vi "VIH Dialog - Find File on Disk.vi"(8 "error in":errorcluster, 9 "File Path":path, 10 "Tree Item Tag":string, 11 "Project Tree":T1) -> (0 "error out":errorcluster, 1 "New File Path":path, 2 "New Tree Item Tag":string, 3 "dup Project Tree":T1)   [LabVIEW 2014]
doc: "::: VI Helpeks :::\nCopyright (c) 2000-2026 Konstantin Shifershteyn. All rights reserved."
uses:
  VIH Project Tree Typedef - Tree Refnum.ctl
panel:
  # "VI Helpeks\nCopyright (c) 2012-2026 Konstantin Shifershteyn"
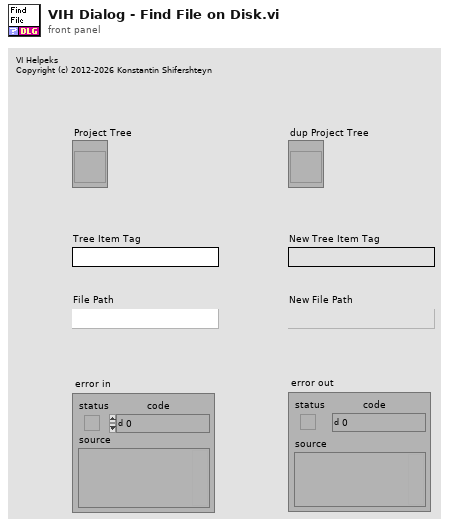
[diagram p1: front panel]
types:
  T1 = typedef "VIH Project Tree Typedef - Tree Refnum.ctl" = refnum<vi>
  T2 = cluster{"Left Button Key Shortcut":cluster{"Control":bool, "Shift":bool, "Key":string}, "Center Button Key Shortcut":cluster{"Control":bool, "Shift":bool, "Key":string}, "Right Button Key Shortcut":cluster{"Control":bool, "Shift":bool, "Key":string}}
  T3 = enum16{"Left Button", "Center Button", "Right Button", "Window Close"}
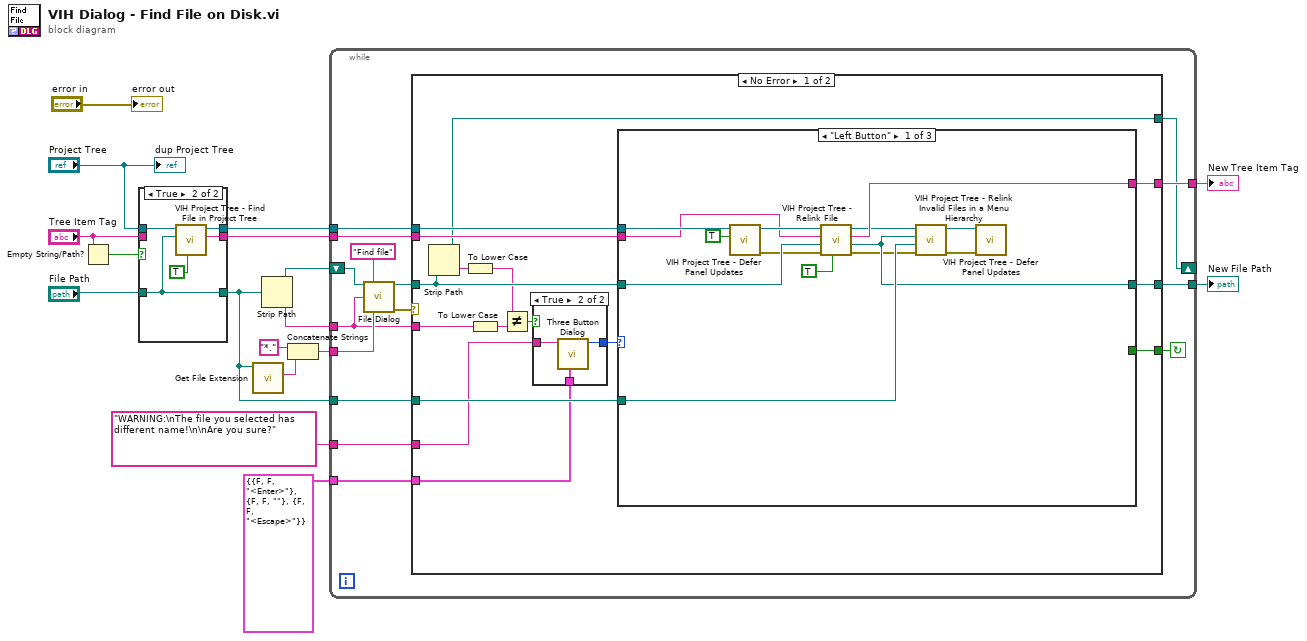
[diagram p0: block diagram]
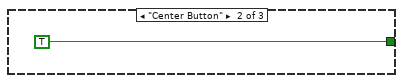
[diagram p2: hidden frame]
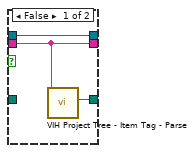
[diagram p6: hidden frame]
diagram:
  n1 = Empty String/Path?(string/path="Tree Item Tag") -> (empty?=w15:bool)
  n2 = case shown="True" w15 {
    tunnel: [w20 w24] -> w5
    tunnel: "Tree Item Tag" -> [w19 _]
    tunnel: [w19 w25] -> w14
    tunnel: "File Path" -> [_ w24]
    tunnel: "Project Tree" -> [w18 w23]
    tunnel: [w18 w21] -> w7
    frame False {
      n3 = call "VIH Project Tree - Item Tag - Parse.vi"("Tree Item Tag"=w19) -> ("Item File Path"=w20:path)  [unwired: 8 in, 2 out]
    }
    frame True {
      n4 = call "VIH Project Tree - Find File in Project Tree.vi"("Ena <Invalid> (F)"=TRUE, "File Path"=w24, "Project Tree"=w23) -> ("Tree Item Tag (Static)"=w25:string, "dup Project Tree"=w21:T1)  [unwired: 5 in, 2 out]
    }
  }
  n5 = call <vilib>:"Get File Extension.vi"("file"=w5) -> ("lowercase file extension"=w2:string)  [unwired: 7 in, 3 out]
  n6 = Strip Path(path=w5) -> (stripped path=w1:path, name=w3:string)
  n7 = Concatenate Strings("*." ("string"), w2) -> (w4:string)
  n8 = while {
    tunnel: w14 -> [w37]
    tunnel: [w36] -> w11
    tunnel: [w35] -> w10
    tunnel: "WARNING:\nThe file you selected has different name!\n\nAre you sure?" ("message") -> [w34]
    tunnel: T2 {"Left Button Key Shortcut"={"Control"=FALSE, "Shift"=FALSE, "Key"="<Enter>"}, "Center Button Key Shortcut"={"Control"=FALSE, "Shift"=FALSE, "Key"=""}, "Right Button Key Shortcut"={"Control"=FALSE, "Shift"=FALSE, "Key"="<Escape>"}} ("Keyboard Shortcuts (Left is <Enter>)") -> [w33]
    tunnel: w7 -> [w32]
    tunnel: w5 -> [w30]
    tunnel: w4 -> [w29]
    tunnel: w3 -> [w28]
    shift-right: [w26] -> _
    shift-left: w1 -> [w27]
    stop <- w31 continue-if-true
    n9 = call "File Dialog"("start path"=w27, "prompt"="Find file", "default name"=w28, "pattern (all files)"=w29) -> ("selected path"=w40:path, "error out"=w39:errorcluster)  [unwired: 8 in, 2 out]
    n10 = case shown="No Error" w39 {
      tunnel: w32 -> [w56 _]
      tunnel: w37 -> [w55 _]
      tunnel: w40 -> [w51 _]
      tunnel: w30 -> [w54 _]
      tunnel: [w53 _] -> w36
      tunnel: [w52 _] -> w35
      tunnel: w28 -> [w47 _]
      tunnel: w34 -> [w45 _]
      tunnel: w33 -> [w44 _]
      tunnel: [w42 _] -> w31
      tunnel: [w41 _] -> w26
      frame No Error {
        n11 = Strip Path(path=w51) -> (stripped path=w41:path, name=w50:string)
        n12 = To Lower Case(string=w50) -> (all lower case string=w49:string)
        n13 = To Lower Case(string=w47) -> (all lower case string=w48:string)
        n14 = Not Equal?(x=w49, y=w48) -> (x != y?=w46:bool)
        n15 = case shown="True" w46 {
          tunnel: w45 -> [_ w74]
          tunnel: w44 -> [_ w73]
          tunnel: [_ w72] -> w43
          frame False {
          }
          frame True {
            n16 = call <vilib>:"Three Button Dialog.vi"("Keyboard Shortcuts (Left is <Enter>)"=w73, "message"=w74) -> ("Which Button?"=w72:T3)  [unwired: 9 in]
          }
        }
        n17 = case shown="\"Left Button\"" w43 {
          tunnel: w56 -> [w63 _ _]
          tunnel: w55 -> [w57 _ _]
          tunnel: w54 -> [w70 _ _]
          tunnel: [w68 _ _] -> w53
          tunnel: [w67 _ _] -> w52
          tunnel: w51 -> [w69 _ _]
          tunnel: [_ TRUE _] -> w42
          frame "Left Button" {
            n18 = call "VIH Project Tree - Defer Panel Updates.vi"("Defer Panel Updates (F)"=TRUE, "Project Tree"=w63) -> ("error out"=w60:errorcluster, "dup Project Tree"=w62:T1)  [unwired: 7 in, 1 out]
            n19 = call "VIH Project Tree - Relink File.vi"("Ena Dialog Message (T)"=TRUE, "error in"=w60, "New File Path"=w69, "Tree Item Tag"=w57, "Project Tree"=w62) -> ("error out"=w64:errorcluster, "New File Path out"=w67:path, "New Tree Item Tag"=w68:string, "dup Project Tree"=w66:T1)  [unwired: 3 in]
            n20 = call "VIH Project Tree - Relink Invalid Files in a Menu Hierarchy.vi"("error in"=w64, "old Item Path"=w70, "new Item Path"=w67, "Project Tree"=w66) -> ("error out"=w59:errorcluster, "dup Project Tree"=w61:T1)  [unwired: 6 in]
            n21 = call "VIH Project Tree - Defer Panel Updates.vi"("error in"=w59, "Project Tree"=w61) -> ()  [unwired: 7 in, 3 out]
          }
          frame "Center Button" {
          }
          frame "Right Button", "Window Close" {
          }
        }
      }
      frame Error {
      }
    }
  }
  "New Tree Item Tag" <- w11
  "New File Path" <- w10
  "dup Project Tree" <- "Project Tree"
  "error out" <- "error in"
